vi "Demande Acquisition.vi"() -> ()   [LabVIEW 2022 SP3]
uses:
  Enum/Enum 4.ctl
  Enum/Enum 5.ctl
  Variables globales/Variable glob Pt.vi
  Variables globales/Variable glob Leybold.vi
  Variables globales/Variable glob Edwards.vi
  Variables globales/Variable glob Keller.vi
  Variables globales/Variable glob Th.vi
  Variables globales/Variables glob EUROTHERM.vi
  Variables globales/Variable globale compteurs.vi
  Variables globales/Variable glob generale.vi
  Variables globales/Variable glob mails.vi
  Variables globales/Variable glob alertes ecart temperatures.vi
  Variables globales/Variable glob alertes min-max temperatures.vi
  Variables globales/Variable glob alertes pressions.vi
  Variables globales/Variable glob alertes Keller.vi
  Variables globales/Variable glob alertes Compteurs.vi
panel:
  out "message":string="LANCEMENT DES ACQUISITIONS EN COURS"
  out "référence au VI":refnum<vi>
  out "sortie d'erreur":errorcluster
  in  "Annuler":bool
  in  "Commande onglets":T1(tab)
  out "Liste mails":string[](array[string]) caption="Liste mails envoi alarmes"
  out "Entête du fichier":string
  out "Dossier du fichier sauvegarde :":path
  out "Dossier du fichier distant :":path
  out "Dossier du fichier local :":path
  out "Nom des pressions LEYBOLD sélectionnées":string[](array[string])
  out "Nom des pressions EDWARDS sélectionnées":string[](array[string])
  out "Nom des pressions KELLER sélectionnées":string[](array[string])
  out "Nom des thermocouples sélectionnés":string[](array[string])
  out "Nom des platines sélectionnées :":string[](array[string])
  out "Régulateurs EUROTHERM sélectionnés":string[](array[string])
  out "Intervale de temps (s) pour débit":u16
  out "Nom des compteurs GN2 sélectionnées :":string[](array[string])
  in  "OK":bool
  in  "Lancement":bool caption="Arrêt"
  # "Lancement/arrêt des acquisitions\ntempératures, pressions, eurotherm,\nkeller et compteurs"
  # "Ce logiciel et les informations qu'il contient, sont la propriété de l’IAS et ne peuvent être diffusés sans l’autorisation de la Station d’étalonnage"
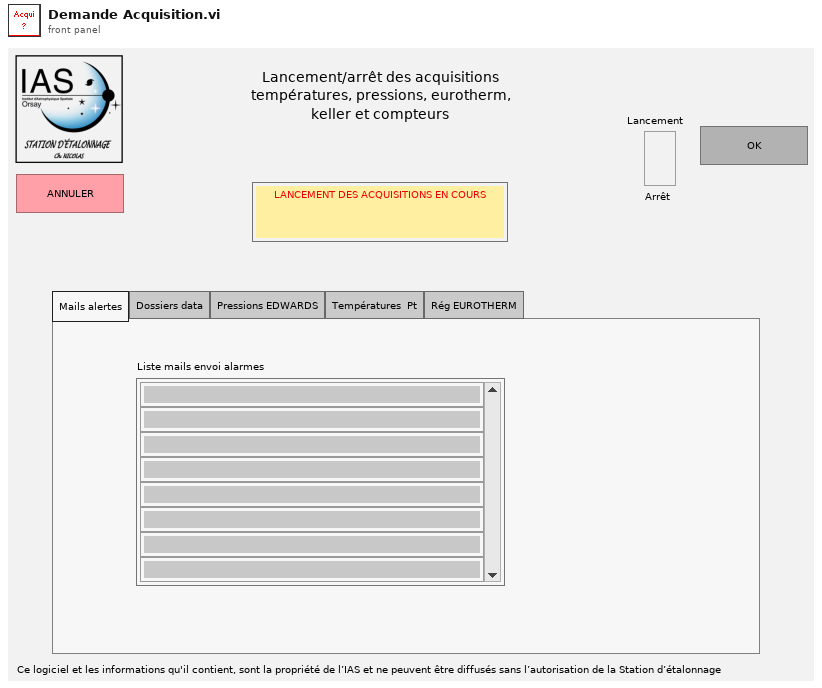
[diagram p1: front panel]
types:
  T1 = enum32{"Mails alertes", "Dossiers data", "Pressions LEYBOLD", "Pressions EDWARDS", "Pressions KELLER", "Températures Th", "Températures  Pt", "Rég EUROTHERM", "COMPTEURS"}
  T2 = typedef "Enum 4.ctl" = enum16{"Init var locales", "Init pages", "Init noms", "Confirmation", "Lancement", "Arrêt", "Fin"}
  T3 = typedef "Enum 5.ctl" = enum16{"nom manip", "lancement", "acqui", "tempo", "surveillance alarme reg", "enregistrement local", "enregistrement distant", "enregistrement sauvegarde", "erreur", "fin"}
  T4 = enum32{"Invalid", "Standard", "Closed", "Hidden", "Minimized", "Maximized"}
  T5 = cluster{"Noms voies select acqui 1COM":string[]}[]
  T6 = cluster{"Nom tache Pt":refnum<k21>, "Noms des Pt":string[], "Nb Pt":i16, "Selection Pt":bool[], "Nom Pt selectionnees":string[]}[]
  T7 = cluster{"Nom tache compteurs":refnum<k21>, "Noms des compteurs":string[], "Selection":bool[], "Init compteurs":dbl[], "Noms compteurs selectionnes":string[]}
  T8 = cluster{"Nom tache Th":refnum<k21>, "Noms des Th":string[], "Nb Th":i16, "Selection Th":bool[], "Nom Th selectionnes":string[]}[]
  T9 = cluster{"Indices a controler":i16[], "Defaut":bool, "ecart temp":dbl, "Alerte":bool, ">?":bool, "N°":u16}[]
  T10 = cluster{"Alerte temp min/max":bool, "température max":dbl, "température min":dbl, "Défaut min/max temp":bool, "Indices à controler":i16[], "N°":u16}[]
  T11 = cluster{"Alerte Keller":bool, "valeur alerte Keller":dbl, "Défaut Keller":bool, "Indices Keller à controler":i16[], "N°":u16}[]
  T12 = cluster{"Alerte Keller":bool, "valeur alerte Keller":dbl, "Défaut Keller":bool, "Indices Keller à controler":i16[], "N°":u16}
  T13 = cluster{"Indices a controler":i16[], "Defaut":bool, "ecart temp":dbl, "Alerte":bool, ">?":bool, "N°":u16}
  T14 = cluster{"Alerte temp min/max":bool, "température max":dbl, "température min":dbl, "Défaut min/max temp":bool, "Indices à controler":i16[], "N°":u16}
  T15 = cluster{"Alerte":bool, "valeur alerte":dbl, "Défaut":bool, "Indices à controler":i16[], "N°":u16}[]
  T16 = cluster{"Alerte":bool, "valeur ":dbl, "Défaut":bool, "Indices controler":i16[], "N°":u16}[]
  T17 = cluster{"Alerte":bool, "valeur alerte":dbl, "Défaut":bool, "Indices à controler":i16[], "N°":u16}
  T18 = cluster{"Alerte":bool, "valeur ":dbl, "Défaut":bool, "Indices controler":i16[], "N°":u16}
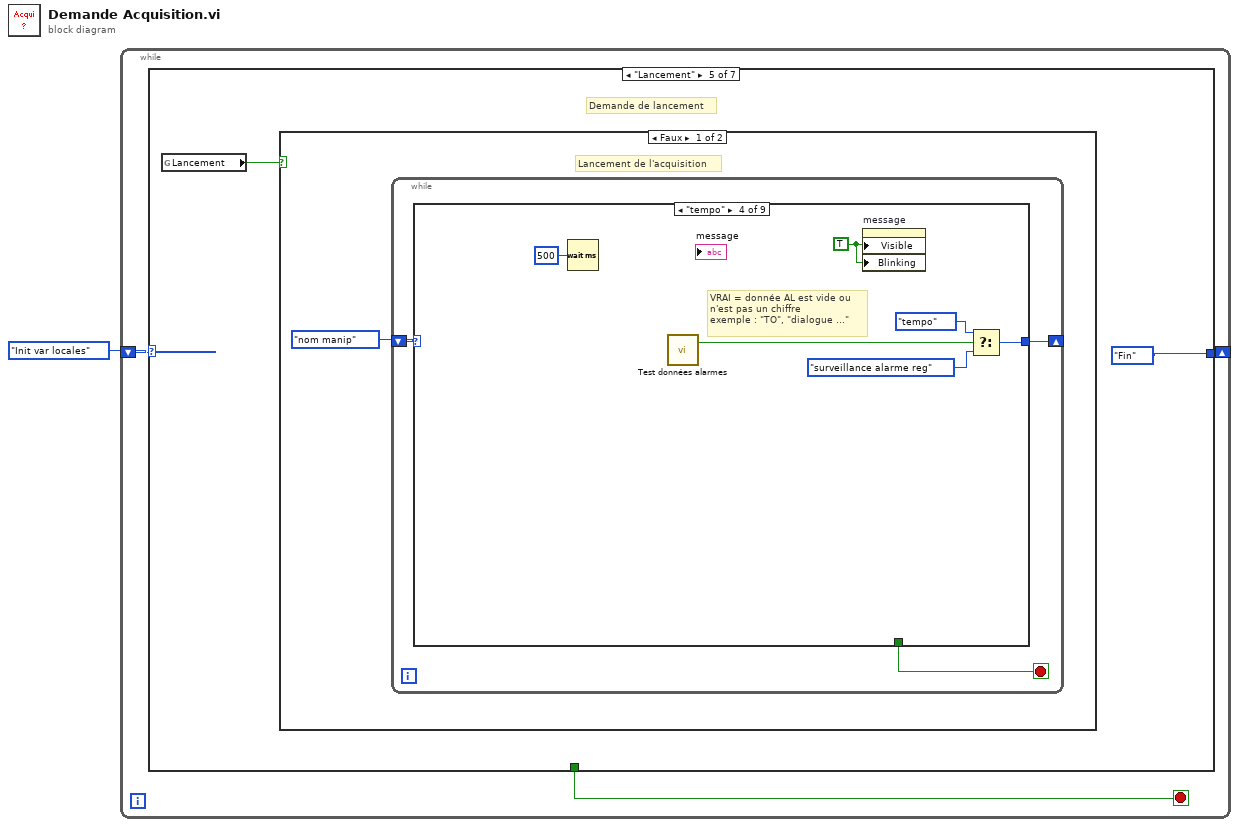
[diagram p0: block diagram]
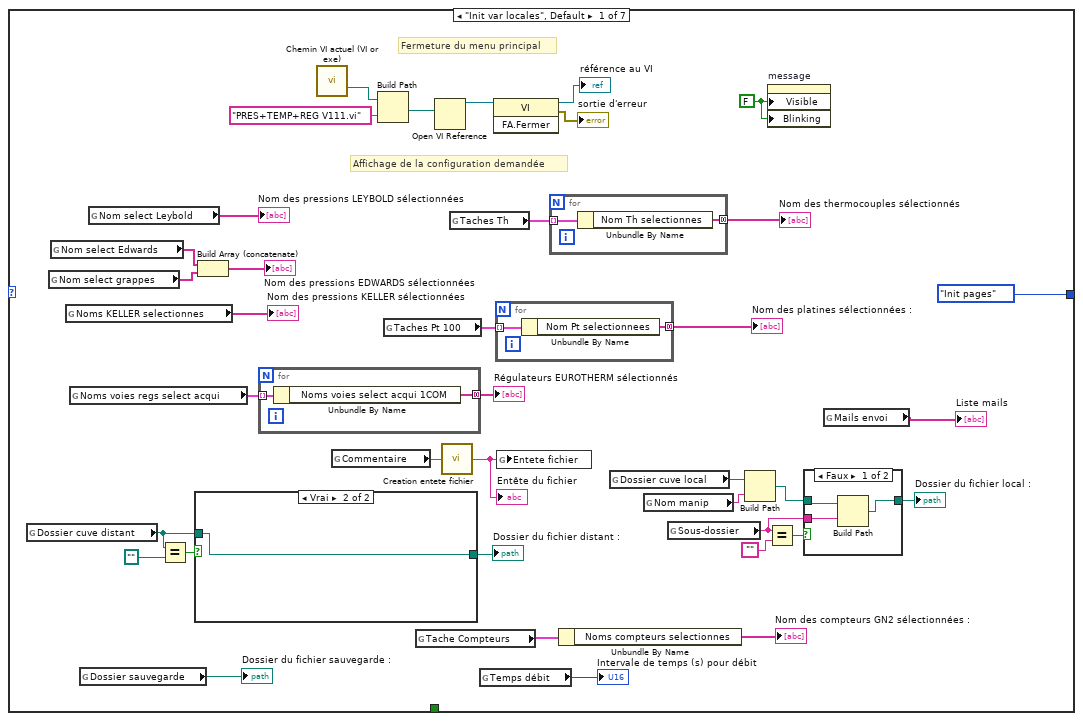
[diagram p2: hidden frame]
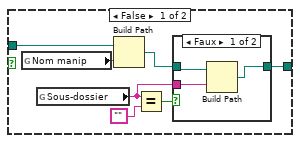
[diagram p3: hidden frame]
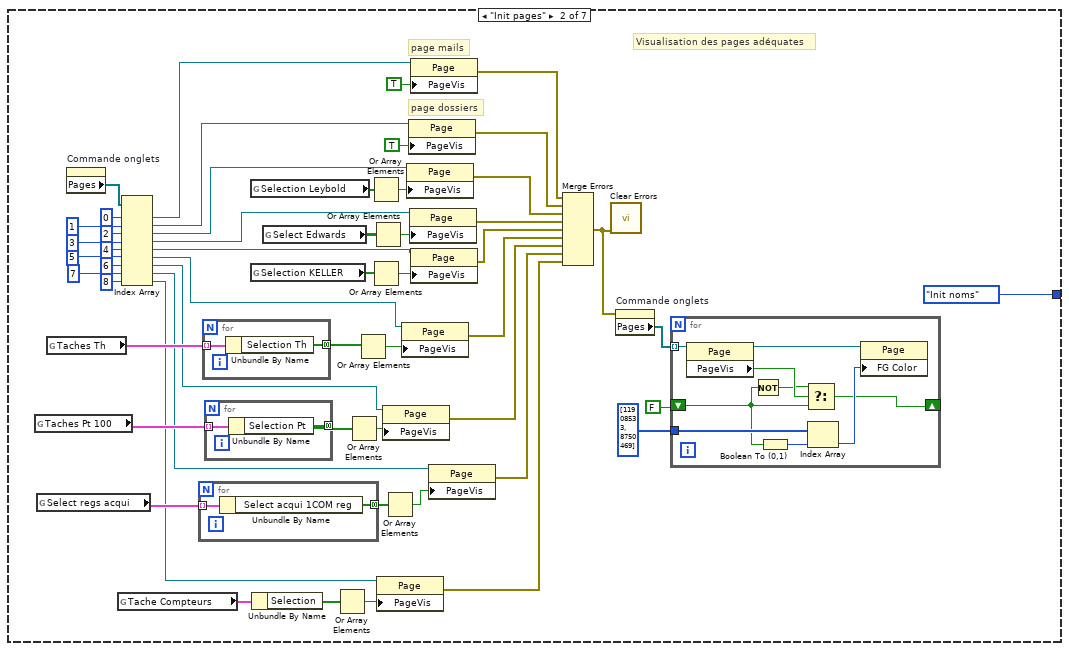
[diagram p6: hidden frame]
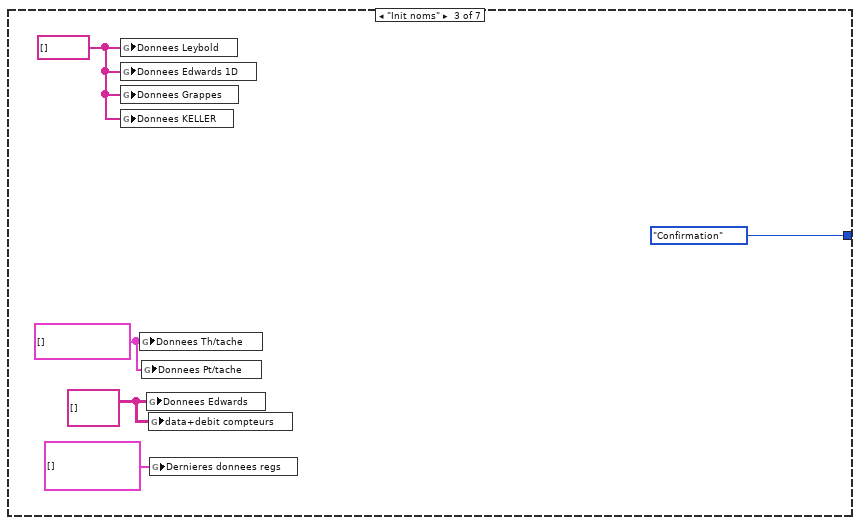
[diagram p7: hidden frame]
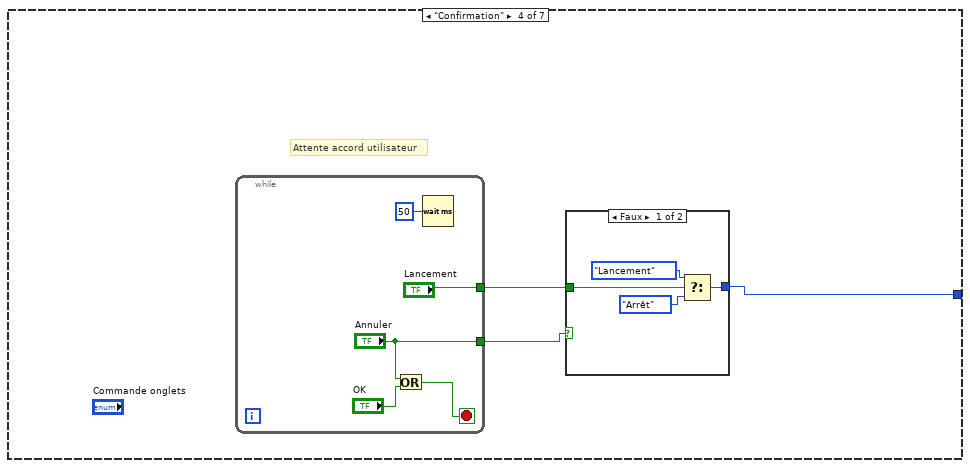
[diagram p8: hidden frame]
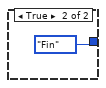
[diagram p9: hidden frame]
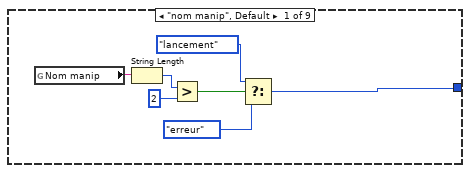
[diagram p10: hidden frame]
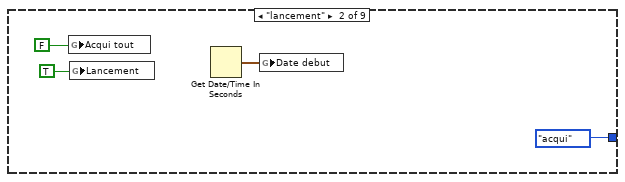
[diagram p11: hidden frame]
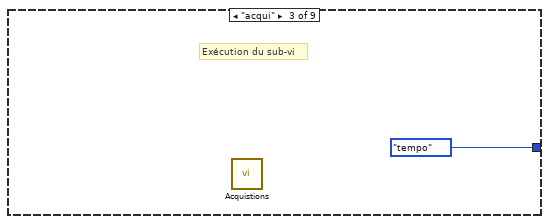
[diagram p12: hidden frame]
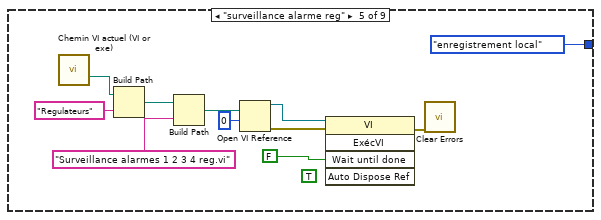
[diagram p13: hidden frame]
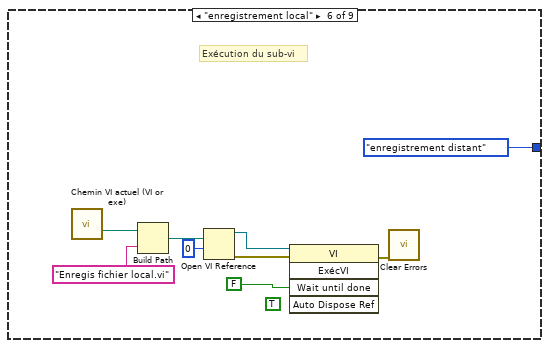
[diagram p14: hidden frame]
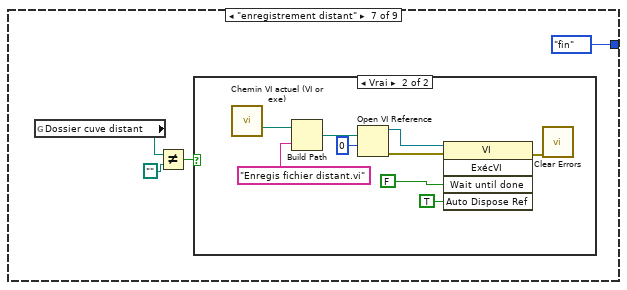
[diagram p15: hidden frame]
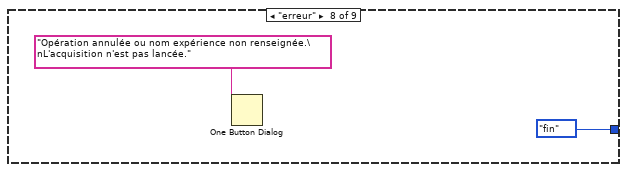
[diagram p17: hidden frame]
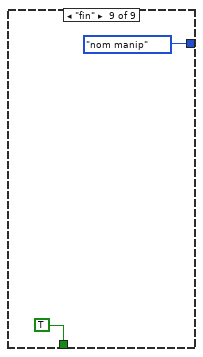
[diagram p18: hidden frame]
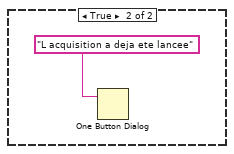
[diagram p19: hidden frame]
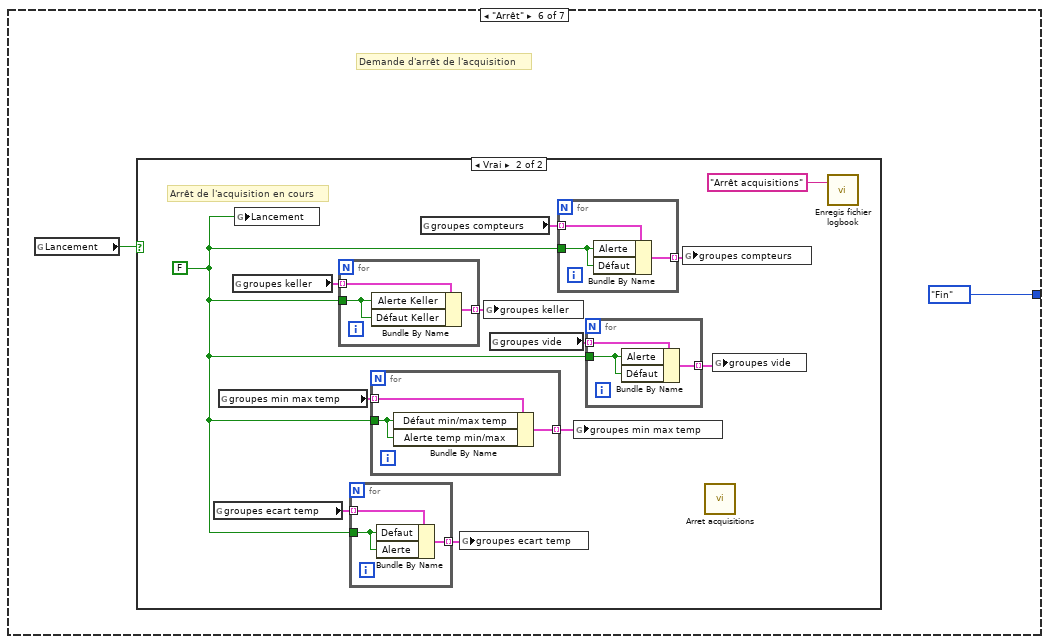
[diagram p20: hidden frame]
diagram:
  n1 = while {
    shift-right: [w3] -> _
    shift-left: Enum_4."Init var locales" ("Énum") -> [w4]
    stop <- w2 stop-if-true
    n2 = case shown="\"Lancement\"" w4 {
      tunnel: [Enum_4."Init pages" ("Énum") Enum_4."Init noms" ("Énum") Enum_4."Confirmation" ("Énum") w138 Enum_4."Fin" ("Énum") Enum_4."Fin" ("Énum") Enum_4."Init pages" ("Énum")] -> w3
      tunnel: [_ _ _ _ _ _ TRUE] -> w2
      frame "Init var locales", Default {
        w23 = FALSE ("Visible")
        # "Affichage de la configuration demandée"
        # "Fermeture du menu principal"
        n3 = global read "Variable glob generale.vi" "Dossier cuve distant"() -> (w7:path)
        n4 = global read "Variable glob Edwards.vi" "Nom select grappes"() -> (w32:string[])
        n5 = global read "Variable glob Edwards.vi" "Nom select Edwards"() -> (w33:string[])
        n6 = global read "Variable glob Keller.vi" "Noms KELLER selectionnes"() -> (→"Nom des pressions KELLER sélectionnées":string[])
        n7 = global read "Variables glob EUROTHERM.vi" "Noms voies regs select acqui"() -> (w25:T5)
        n8 = global read "Variable glob generale.vi" "Dossier sauvegarde"() -> (→"Dossier du fichier sauvegarde :":path)
        n9 = global read "Variable glob Leybold.vi" "Nom select Leybold"() -> (→"Nom des pressions LEYBOLD sélectionnées":string[])
        n10 = Equal?(x=w7, y=path "") -> (x = y?=w8:bool)
        n11 = case shown="Vrai" w8 {
          tunnel: [w43 w53] -> w9
          tunnel: w7 -> [w42 w53]
          frame False {
            n12 = global read "Variable glob generale.vi" "Nom manip"() -> (w44:string)
            n13 = global read "Variable glob generale.vi" "Sous-dossier"() -> (w47:string)
            n14 = Build Path(base path=w42, name or relative path=w44) -> (appended path=w48:path)
            n15 = Equal?(x=w47, y="") -> (x = y?=w45:bool)
            n16 = case shown="Faux" w45 {
              tunnel: w47 -> [w51 _]
              tunnel: w48 -> [w50 w52]
              tunnel: [w49 w52] -> w43
              frame False {
                n17 = Build Path(base path=w50, name or relative path=w51) -> (appended path=w49:path)
              }
              frame True {
              }
            }
          }
          frame True {
          }
        }
        "Dossier du fichier distant :" <- w9
        n18 = Build Array (concatenate)(w33, w32) -> (→"Nom des pressions EDWARDS sélectionnées":string[])
        n19 = for {
          tunnel: w25 -> [w59] mode=indexing
          tunnel: [w58] -> w24 mode=concatenating
          n20 = Unbundle By Name(w59) -> ("Noms voies select acqui 1COM"=w58:string[])
        }
        "Régulateurs EUROTHERM sélectionnés" <- w24
        n21 = call "Chemin VI actuel (VI or exe).vi"() -> ("VI or executable installation directory"=w30:path)  [unwired: 14 in, 1 out]
        n22 = global read "Variable glob generale.vi" "Commentaire"() -> (w18:string)
        n23 = Build Path(base path=w30, name or relative path="PRES+TEMP+REG V111.vi" ("nom ou chemin relatif")) -> (appended path=w35:path)
        n24 = global read "Variable glob Pt.vi" "Taches Pt 100"() -> (w29:T6)
        n25 = global read "Variable globale compteurs.vi" "Tache Compteurs"() -> (w22:T7)
        n26 = Open VI Reference(vi path=w35) -> (vi reference=w34:refnum<vi>)  [unwired: 5 in, 1 out]
        n27 = call "Creation entete fichier.vi"("Commentaire"=w18) -> ("Entête fichier"=w17:string)
        "Entête du fichier" <- w17
        n28 = global read "Variable glob Th.vi" "Taches Th"() -> (w27:T8)
        n29 = global read "Variable globale compteurs.vi" "Temps débit"() -> (→"Intervale de temps (s) pour débit":u16)
        n30 = invoke class="VI" method="FA.Fermer"(reference=w34) -> (reference out=→"référence au VI":refnum<vi>, error out=→"sortie d'erreur":errorcluster)  [unwired: 2 in, 1 out]
        n31 = for {
          tunnel: w29 -> [w63] mode=indexing
          tunnel: [w62] -> w28 mode=concatenating
          n32 = Unbundle By Name(w63) -> ("Nom Pt selectionnees"=w62:string[])
        }
        "Nom des platines sélectionnées :" <- w28
        n33 = global write "Variable glob generale.vi" "Entete fichier"(w17) -> ()
        n34 = for {
          tunnel: w27 -> [w61] mode=indexing
          tunnel: [w60] -> w26 mode=concatenating
          n35 = Unbundle By Name(w61) -> ("Nom Th selectionnes"=w60:string[])
        }
        "Nom des thermocouples sélectionnés" <- w26
        n36 = Unbundle By Name(w22) -> ("Noms compteurs selectionnes"=→"Nom des compteurs GN2 sélectionnées :":string[])
        n37 = global read "Variable glob generale.vi" "Dossier cuve local"() -> (w16:path)
        n38 = global read "Variable glob generale.vi" "Nom manip"() -> (w15:string)
        n39 = global read "Variable glob generale.vi" "Sous-dossier"() -> (w12:string)
        n40 = Build Path(base path=w16, name or relative path=w15) -> (appended path=w11:path)
        n41 = Equal?(x=w12, y="") -> (x = y?=w14:bool)
        n42 = property on="message" class="Ch"("Visible"=w23, "Blinking"=w23) -> ()  [unwired: 2 in, 2 out]
        n43 = case shown="Faux" w14 {
          tunnel: w12 -> [w56 _]
          tunnel: w11 -> [w55 w57]
          tunnel: [w54 w57] -> w10
          frame False {
            n44 = Build Path(base path=w55, name or relative path=w56) -> (appended path=w54:path)
          }
          frame True {
          }
        }
        "Dossier du fichier local :" <- w10
        n45 = global read "Variable glob mails.vi" "Mails envoi"() -> (→"Liste mails":string[])
      }
      frame "Init pages" {
        # "page dossiers"
        # "page mails"
        # "Visualisation des pages adéquates"
        n46 = global read "Variable glob Pt.vi" "Taches Pt 100"() -> (w92:T6)
        n47 = global read "Variables glob EUROTHERM.vi" "Select regs acqui"() -> (w88:cluster{"Select acqui 1COM reg":bool[]}[])
        n48 = global read "Variable glob Th.vi" "Taches Th"() -> (w90:T8)
        n49 = property on="Commande onglets" class="Onglet (strict)"() -> ("Pages"=w107:refnum<vi>[])  [unwired: 2 in, 2 out]
        n50 = global read "Variable globale compteurs.vi" "Tache Compteurs"() -> (w77:T7)
        n51 = Index Array(array=w107, index #1=0 ("indice"), index #2=1 ("indice"), index #3=2 ("indice"), index #4=3 ("indice"), index #5=4 ("indice"), index #6=5 ("indice"), index #7=6 ("indice"), index #8=7 ("indice"), index #9=8 ("indice")) -> (element #1=w86:refnum<vi>, element #2=w72:refnum<vi>, element #3=w71:refnum<vi>, element #4=w70:refnum<vi>, element #5=w69:refnum<vi>, element #6=w68:refnum<vi>, element #7=w67:refnum<vi>, element #8=w66:refnum<vi>, element #9=w65:refnum<vi>)
        n52 = for {
          tunnel: w88 -> [w127] mode=indexing
          tunnel: [w126] -> w87 mode=concatenating
          n53 = Unbundle By Name(w127) -> ("Select acqui 1COM reg"=w126:bool[])
        }
        n54 = for {
          tunnel: w90 -> [w129] mode=indexing
          tunnel: [w128] -> w89 mode=concatenating
          n55 = Unbundle By Name(w129) -> ("Selection Th"=w128:bool[])
        }
        n56 = for {
          tunnel: w92 -> [w131] mode=indexing
          tunnel: [w130] -> w91 mode=concatenating
          n57 = Unbundle By Name(w131) -> ("Selection Pt"=w130:bool[])
        }
        n58 = global read "Variable glob Leybold.vi" "Selection Leybold"() -> (w104:bool[])
        n59 = global read "Variable glob Keller.vi" "Selection KELLER"() -> (w113:bool[])
        n60 = Unbundle By Name(w77) -> ("Selection"=w76:bool[])
        n61 = global read "Variable glob Edwards.vi" "Select Edwards"() -> (w106:bool[][])
        n62 = Or Array Elements(Boolean array=w76) -> (logical OR=w78:bool)
        n63 = Or Array Elements(Boolean array=w91) -> (logical OR=w115:bool)
        n64 = Or Array Elements(Boolean array=w89) -> (logical OR=w114:bool)
        n65 = Or Array Elements(Boolean array=w104) -> (logical OR=w105:bool)
        n66 = Or Array Elements(Boolean array=w113) -> (logical OR=w102:bool)
        n67 = Or Array Elements(Boolean array=w106) -> (logical OR=w103:bool)
        n68 = property class="Page"(reference=w65, "PageVis"=w78) -> (error out=w75:errorcluster)  [unwired: 1 in, 1 out]
        n69 = property class="Page"(reference=w67, "PageVis"=w115) -> (error out=w100:errorcluster)  [unwired: 1 in, 1 out]
        n70 = Or Array Elements(Boolean array=w87) -> (logical OR=w96:bool)
        n71 = property class="Page"(reference=w68, "PageVis"=w114) -> (error out=w99:errorcluster)  [unwired: 1 in, 1 out]
        n72 = property class="Page"(reference=w71, "PageVis"=w105) -> (error out=w101:errorcluster)  [unwired: 1 in, 1 out]
        n73 = property class="Page"(reference=w72, "PageVis"=TRUE ("Page visible")) -> (error out=w64:errorcluster)  [unwired: 1 in, 1 out]
        n74 = property class="Page"(reference=w70, "PageVis"=w103) -> (error out=w98:errorcluster)  [unwired: 1 in, 1 out]
        n75 = property class="Page"(reference=w86, "PageVis"=TRUE ("Page visible")) -> (error out=w84:errorcluster)  [unwired: 1 in, 1 out]
        n76 = property class="Page"(reference=w69, "PageVis"=w102) -> (error out=w97:errorcluster)  [unwired: 1 in, 1 out]
        n77 = property class="Page"(reference=w66, "PageVis"=w96) -> (error out=w95:errorcluster)  [unwired: 1 in, 1 out]
        n78 = Merge Errors(w84, w64, w101, w98, w97, w99, w100, w95, w75) -> (w81:errorcluster)
        n79 = call <vilib>:"Clear Errors.vi"("error in (no error)"=w81) -> ()  [unwired: 5 in, 2 out]
        n80 = property on="Commande onglets" class="Onglet (strict)"(error in=w81) -> ("Pages"=w80:refnum<vi>[])  [unwired: 1 in, 2 out]
        n81 = for {
          tunnel: w80 -> [w125] mode=indexing
          tunnel: u32[] [11908533, 8750469] ("Tableau") -> [w122]
          shift-right: [w117] -> _
          shift-left: FALSE -> [w118]
          n82 = property class="Page"(reference=w125) -> (reference out=w124:refnum<vi>, "PageVis"=w123:bool)  [unwired: 1 in, 1 out]
          n83 = Not(x=w118) -> (.not. x?=w119:bool)
          n84 = Boolean To (0,1)(Boolean=w118) -> (0, 1=w120:i16)
          n85 = Select(t=w119, s=w123, f=w118) -> (s? t:f=w117:bool)
          n86 = Index Array(array=w122, index=w120) -> (element=w121:u32)
          n87 = property class="Page"(reference=w124, "FG Color"=w121) -> ()  [unwired: 1 in, 2 out]
        }
      }
      frame "Init noms" {
        w135 = cluster{"Données Th":string[]}[] [] ("Données Th/tache")
        w132 = string[][] [] ("Données Edwards")
        w133 = string[] [] ("Données Leybold")
        n88 = global write "Variable glob Leybold.vi" "Donnees Leybold"(w133) -> ()
        n89 = global write "Variable glob Edwards.vi" "Donnees Edwards 1D"(w133) -> ()
        n90 = global write "Variable glob Edwards.vi" "Donnees Grappes"(w133) -> ()
        n91 = global write "Variable glob Keller.vi" "Donnees KELLER"(w133) -> ()
        n92 = global write "Variable glob Th.vi" "Donnees Th/tache"(w135) -> ()
        n93 = global write "Variable glob Pt.vi" "Donnees Pt/tache"(w135) -> ()
        n94 = global write "Variable glob Edwards.vi" "Donnees Edwards"(w132) -> ()
        n95 = global write "Variable globale compteurs.vi" "data+debit compteurs"(w132) -> ()
        n96 = global write "Variables glob EUROTHERM.vi" "Dernieres donnees regs"(cluster{"Dernières données 1COM":string[][]}[] [] ("Dernières données regs")) -> ()
      }
      frame "Confirmation" {
        # "Attente accord utilisateur"
        n97 = while {
          tunnel: ["Lancement"] -> w139
          tunnel: ["Annuler"] -> w137
          stop <- w147 stop-if-true
          n98 = Or(x="Annuler", y="OK") -> (x .or. y?=w147:bool)
          n99 = Wait (ms)(milliseconds to wait=u32 50 ("attente (ms)")) -> ()  [unwired: 1 out]
        }
        n100 = case shown="Faux" w137 {
          tunnel: w139 -> [w143 _]
          tunnel: [w140 Enum_4."Fin" ("Énum")] -> w138
          frame False {
            n101 = Select(t=Enum_4."Lancement" ("Énum"), s=w143, f=Enum_4."Arrêt" ("Énum")) -> (s? t:f=w140:T2)
          }
          frame True {
          }
        }
      }
      frame "Lancement" {
        # "Demande de lancement"
        n102 = global read "Variable glob generale.vi" "Lancement"() -> (w151:bool)
        n103 = case shown="Faux" w151 {
          frame False {
            # "Lancement de l'acquisition"
            n104 = while {
              shift-right: [w154] -> _
              shift-left: Enum_5."nom manip" ("Énum") -> [w155]
              stop <- w153 stop-if-true
              n105 = case shown="\"tempo\"" w155 {
                tunnel: [w162 Enum_5."acqui" ("Énum") Enum_5."tempo" ("Énum") w168 Enum_5."enregistrement local" ("Énum") Enum_5."enregistrement distant" ("Énum") Enum_5."fin" ("Énum") Enum_5."fin" ("Énum") Enum_5."nom manip" ("Énum")] -> w154
                tunnel: [_ _ _ _ _ _ _ _ TRUE] -> w153
                frame "nom manip", Default {
                  n106 = global read "Variable glob generale.vi" "Nom manip"() -> (w157:string)
                  n107 = String Length(string=w157) -> (length=w161:i32)
                  n108 = Greater?(x=w161, y=2) -> (0:w156:bool)
                  n109 = Select(t=Enum_5."lancement" ("Énum"), s=w156, f=Enum_5."erreur" ("Énum")) -> (s? t:f=w162:T3)
                }
                frame "lancement" {
                  n110 = global write "Variable glob generale.vi" "Acqui tout"(FALSE) -> ()
                  n111 = global write "Variable glob generale.vi" "Lancement"(TRUE) -> ()
                  n112 = Get Date/Time In Seconds() -> (seconds since 1Jan1904=w164:timestamp)
                  n113 = global write "Variable glob generale.vi" "Date debut"(w164) -> ()
                }
                frame "acqui" {
                  # "Exécution du sub-vi"
                  n114 = call "Acquistions.vi"() -> ()  [unwired: 4 in]
                }
                frame "tempo" {
                  w172 = TRUE ("Visible")
                  # "VRAI = donnée AL est vide ou\nn'est pas un chiffre\nexemple : \"TO\", \"dialogue ...\""
                  n115 = Wait (ms)(milliseconds to wait=u32 500 ("attente (ms)")) -> ()  [unwired: 1 out]
                  n116 = call "Test données alarmes.vi"() -> ("Booléen"=w171:bool)  [unwired: 3 in]
                  n117 = property on="message" class="Ch"("Visible"=w172, "Blinking"=w172) -> ()  [unwired: 2 in, 2 out]
                  n118 = Select(t=Enum_5."tempo" ("Énum"), s=w171, f=Enum_5."surveillance alarme reg" ("Énum")) -> (s? t:f=w168:T3)
                }
                frame "surveillance alarme reg" {
                  (unwired) TRUE ("Supprimer la référence automatiquement")
                  n119 = call "Chemin VI actuel (VI or exe).vi"() -> ("VI or executable installation directory"=w176:path)  [unwired: 14 in, 1 out]
                  n120 = Build Path(base path=w176, name or relative path="Regulateurs" ("nom ou chemin relatif")) -> (appended path=w174:path)
                  n121 = Build Path(base path=w174, name or relative path="Surveillance alarmes 1 2 3 4 reg.vi" ("nom ou chemin relatif")) -> (appended path=w180:path)
                  n122 = Open VI Reference(vi path=w180, options=0) -> (vi reference=w183:refnum<vi>, error out=w181:errorcluster)  [unwired: 4 in]
                  n123 = invoke class="VI" method="ExécVI"(reference=w183, error in=w181, "Wait until done"=FALSE ("ON")) -> (error out=w178:errorcluster)  [unwired: 2 in, 4 out]
                  n124 = call <vilib>:"Clear Errors.vi"("error in (no error)"=w178) -> ()  [unwired: 5 in, 2 out]
                }
                frame "enregistrement local" {
                  (unwired) TRUE ("Supprimer la référence automatiquement")
                  # "Exécution du sub-vi"
                  n125 = call "Chemin VI actuel (VI or exe).vi"() -> ("VI or executable installation directory"=w186:path)  [unwired: 14 in, 1 out]
                  n126 = Build Path(base path=w186, name or relative path="Enregis fichier local.vi" ("nom ou chemin relatif")) -> (appended path=w190:path)
                  n127 = Open VI Reference(vi path=w190, options=0) -> (vi reference=w193:refnum<vi>, error out=w191:errorcluster)  [unwired: 4 in]
                  n128 = invoke class="VI" method="ExécVI"(reference=w193, error in=w191, "Wait until done"=FALSE ("ON")) -> (error out=w187:errorcluster)  [unwired: 2 in, 4 out]
                  n129 = call <vilib>:"Clear Errors.vi"("error in (no error)"=w187) -> ()  [unwired: 5 in, 2 out]
                }
                frame "enregistrement distant" {
                  n130 = global read "Variable glob generale.vi" "Dossier cuve distant"() -> (w196:path)
                  n131 = Not Equal?(x=w196, y=path "") -> (x != y?=w197:bool)
                  n132 = case shown="Vrai" w197 {
                    frame False {
                    }
                    frame True {
                      n133 = call "Chemin VI actuel (VI or exe).vi"() -> ("VI or executable installation directory"=w198:path)  [unwired: 14 in, 1 out]
                      n134 = Build Path(base path=w198, name or relative path="Enregis fichier distant.vi" ("nom ou chemin relatif")) -> (appended path=w201:path)
                      n135 = Open VI Reference(vi path=w201, options=0) -> (vi reference=w206:refnum<vi>, error out=w204:errorcluster)  [unwired: 4 in]
                      n136 = invoke class="VI" method="ExécVI"(reference=w206, error in=w204, "Wait until done"=FALSE ("ON"), "Auto Dispose Ref"=TRUE ("Supprimer la référence automatiquement")) -> (error out=w199:errorcluster)  [unwired: 1 in, 4 out]
                      n137 = call <vilib>:"Clear Errors.vi"("error in (no error)"=w199) -> ()  [unwired: 5 in, 2 out]
                    }
                  }
                }
                frame "erreur" {
                  n138 = One Button Dialog(message="Opération annulée ou nom expérience non renseignée.\nL'acquisition n'est pas lancée.") -> ()  [unwired: 1 in, 1 out]
                }
                frame "fin" {
                }
              }
            }
          }
          frame True {
            n139 = One Button Dialog(message="L acquisition a deja ete lancee") -> ()  [unwired: 1 in, 1 out]
          }
        }
      }
      frame "Arrêt" {
        # "Demande d'arrêt de l'acquisition"
        n140 = global read "Variable glob generale.vi" "Lancement"() -> (w213:bool)
        n141 = case shown="Vrai" w213 {
          frame False {
            n142 = One Button Dialog(message="Il n'y a pas d'acquisition en cours") -> ()  [unwired: 1 in, 1 out]
          }
          frame True {
            w215 = FALSE
            # "Arrêt de l'acquisition en cours"
            n143 = global read "Variable glob alertes ecart temperatures.vi" "groupes ecart temp"() -> (w225:T9)
            n144 = global read "Variable glob alertes min-max temperatures.vi" "groupes min max temp"() -> (w223:T10)
            n145 = global read "Variable glob alertes Keller.vi" "groupes keller"() -> (w219:T11)
            n146 = global write "Variable glob generale.vi" "Lancement"(w215) -> ()
            n147 = for {
              tunnel: w219 -> [w232] mode=indexing
              tunnel: [w231] -> w218 mode=indexing
              tunnel: w215 -> [w230]
              n148 = Bundle By Name(cluster=w232, "Alerte Keller"=w230, "Défaut Keller"=w230) -> (w231:T12)
            }
            n149 = for {
              tunnel: w225 -> [w241] mode=indexing
              tunnel: [w240] -> w224 mode=indexing
              tunnel: w215 -> [w239]
              n150 = Bundle By Name(cluster=w241, "Defaut"=w239, "Alerte"=w239) -> (w240:T13)
            }
            n151 = for {
              tunnel: w223 -> [w238] mode=indexing
              tunnel: [w237] -> w222 mode=indexing
              tunnel: w215 -> [w236]
              n152 = Bundle By Name(cluster=w238, "Défaut min/max temp"=w236, "Alerte temp min/max"=w236) -> (w237:T14)
            }
            n153 = global read "Variable glob alertes Compteurs.vi" "groupes compteurs"() -> (w217:T15)
            n154 = global write "Variable glob alertes ecart temperatures.vi" "groupes ecart temp"(w224) -> ()
            n155 = global write "Variable glob alertes Keller.vi" "groupes keller"(w218) -> ()
            n156 = global read "Variable glob alertes pressions.vi" "groupes vide"() -> (w221:T16)
            n157 = for {
              tunnel: w217 -> [w229] mode=indexing
              tunnel: [w228] -> w216 mode=indexing
              tunnel: w215 -> [w227]
              n158 = Bundle By Name(cluster=w229, "Alerte"=w227, "Défaut"=w227) -> (w228:T17)
            }
            n159 = global write "Variable glob alertes min-max temperatures.vi" "groupes min max temp"(w222) -> ()
            n160 = for {
              tunnel: w221 -> [w235] mode=indexing
              tunnel: [w234] -> w220 mode=indexing
              tunnel: w215 -> [w233]
              n161 = Bundle By Name(cluster=w235, "Alerte"=w233, "Défaut"=w233) -> (w234:T18)
            }
            n162 = global write "Variable glob alertes Compteurs.vi" "groupes compteurs"(w216) -> ()
            n163 = call "Arret acquisitions.vi"() -> ()  [unwired: 12 in]
            n164 = global write "Variable glob alertes pressions.vi" "groupes vide"(w220) -> ()
            n165 = call "Enregis fichier logbook.vi"("Chaîne"="Arrêt acquisitions") -> ()  [unwired: 2 in, 1 out]
          }
        }
      }
      frame "Fin" {
        # "Réouverture du menu principal"
        n166 = local read "référence au VI"() -> (w247:refnum<vi>)
        n167 = local read "sortie d'erreur"() -> (w246:errorcluster)
        n168 = Request Deallocation(TRUE ("flag")) -> ()
        n169 = invoke class="VI" method="FA.Ouvrir"(reference=w247, error in=w246, "Activate"=TRUE ("Activer ?"), "State"=T4."Standard" ("État")) -> (reference out=w245:refnum<vi>, error out=w244:errorcluster)  [unwired: 1 in, 3 out]
        n170 = Close Reference(reference=w245, error in (no error)=w244) -> ()  [unwired: 1 out]
        n171 = control-ref of="ce VI"() -> (w242:refnum<vi>)
        n172 = global write "Variables glob EUROTHERM.vi" "Refnum appel suivi AL"(w242) -> ()
      }
    }
  }
